vi "RT_PRV_AO_Adapter.vi"(8 "error in (no error)":errorcluster={"status"=FALSE, "code"=0, "source"="\"\""}, 10 "calibration":string, 11 "Authorized demand":string) -> (0 "error out":errorcluster={"status"=FALSE, "code"=0, "source"="\"\""}, 2 "status ok":bool, 3 "AO result":string)   [LabVIEW 2026]
doc: "INTENT: Convert PRV command to AO channel. LOGIC: Apply calibrated output scaling and enforce maximum clamp; perform channel write."
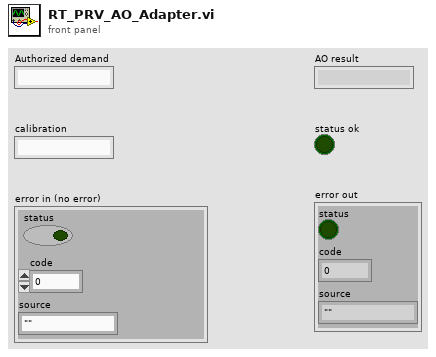
[diagram p1: front panel]
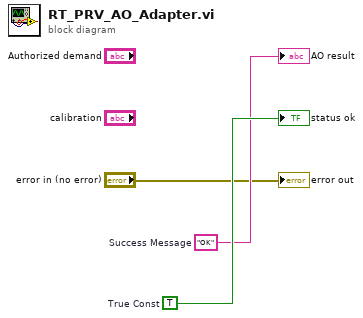
[diagram p0: block diagram]
diagram:
  w3 = TRUE  # True Const
  w2 = "OK"  # Success Message
  "AO result" <- w2
  "status ok" <- w3
  "error out" <- "error in (no error)"
